vi "Log_Part.vi"(8 "error in (no error)":errorcluster, 9 "Line":string, 11 "Log Dir":path) -> (0 "error out":errorcluster)   [LabVIEW 2018]
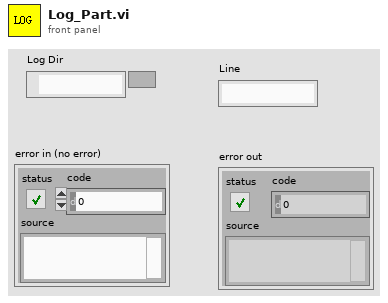
[diagram p1: front panel]
types:
  T1 = enum16{"open", "replace", "create", "open or create", "replace or create", "replace or create with confirmation"}
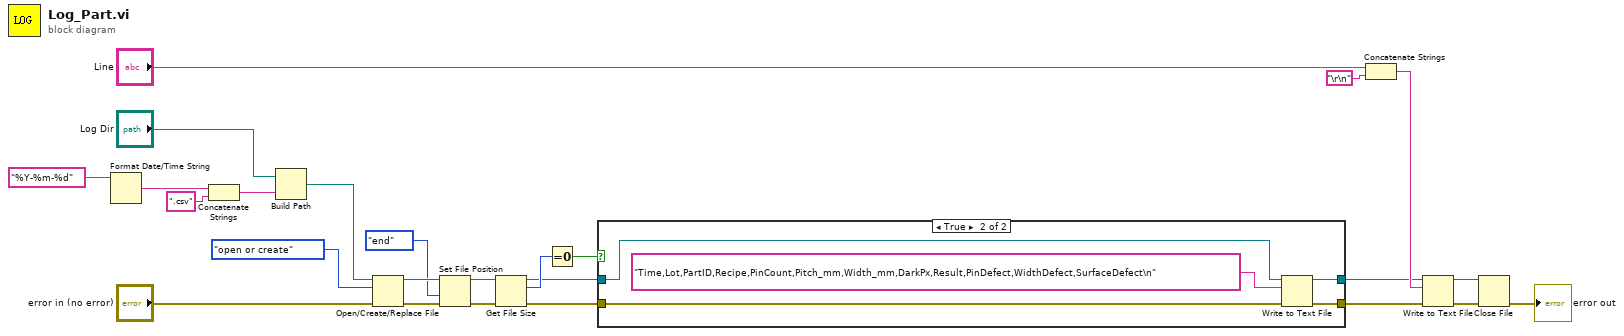
[diagram p0: block diagram]
diagram:
  n1 = Format Date/Time String(time format string (%c)="%Y-%m-%d") -> (date/time string=w24:string)  [unwired: 2 in]
  n2 = Concatenate Strings(w24, ".csv" ("string")) -> (w21:string)
  n3 = Build Path(base path="Log Dir", name or relative path=w21) -> (appended path=w20:path)
  n4 = Open/Create/Replace File(file path (use dialog)=w20, error in="error in (no error)", operation (0:open)=T1."open or create") -> (refnum out=w17:refnum<file>, error out=w16:errorcluster)  [unwired: 3 in, 1 out]
  n5 = Set File Position(refnum=w17, from (0:start)=enum16{"start", "end", "current"}."end", error in=w16) -> (refnum out=w14:refnum<file>, error out=w13:errorcluster)  [unwired: 1 in]
  n6 = Get File Size(file=w14, error in=w13) -> (refnum out=w10:refnum<file>, size (in bytes)=w12:i64, 0:w9:errorcluster)
  n7 = Equal To 0?(x=w12) -> (x = 0?=w11:bool)
  n8 = case shown="True" w11 {
    tunnel: w10 -> [w27 w32]
    tunnel: w9 -> [w26 w31]
    tunnel: [w27 w28] -> w5
    tunnel: [w26 w29] -> w4
    frame False {
    }
    frame True {
      n9 = Write to Text File(file (use dialog)=w32, text="Time,Lot,PartID,Recipe,PinCount,Pitch_mm,Width_mm,DarkPx,Result,PinDefect,WidthDefect,SurfaceDefect\n", error in=w31) -> (refnum out=w28:refnum<file>, error out=w29:errorcluster)  [unwired: 1 in, 1 out]
    }
  }
  n10 = Concatenate Strings("Line", "\r\n") -> (w6:string)
  n11 = Write to Text File(file (use dialog)=w5, text=w6, error in=w4) -> (refnum out=w3:refnum<file>, error out=w2:errorcluster)  [unwired: 1 in, 1 out]
  n12 = Close File(refnum=w3, error in=w2) -> (error out=→"error out":errorcluster)  [unwired: 1 out]
